vi "set Swept SA - Marker.vi"(6 "On?":bool, 8 "error in (no error)":errorcluster, 9 "trace":i32, 10 "Index":i32, 11 "FSV-40N in":refnum<class "FSV-40N.lvclass">) -> (0 "error out":errorcluster, 3 "FSV-40N out":refnum<class "FSV-40N.lvclass">)   [LabVIEW 2023, in "Spectrum Analyzer.lvlib" / "FSV-40N.lvclass"]
uses:
  FSV-40N.lvclass
  FSV-40N.lvclass/FSV-40N.ctl
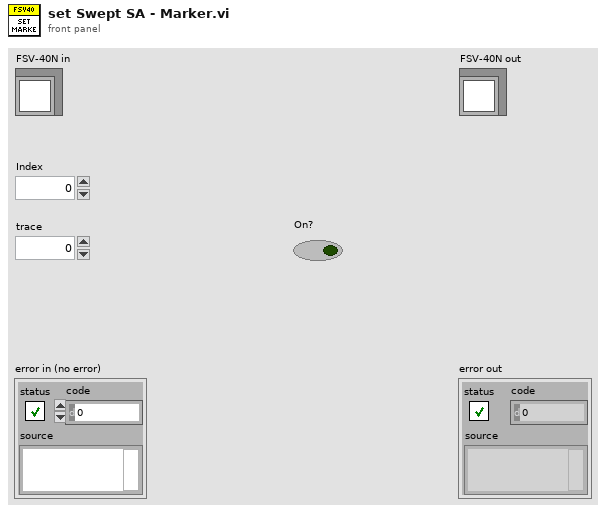
[diagram p1: front panel]
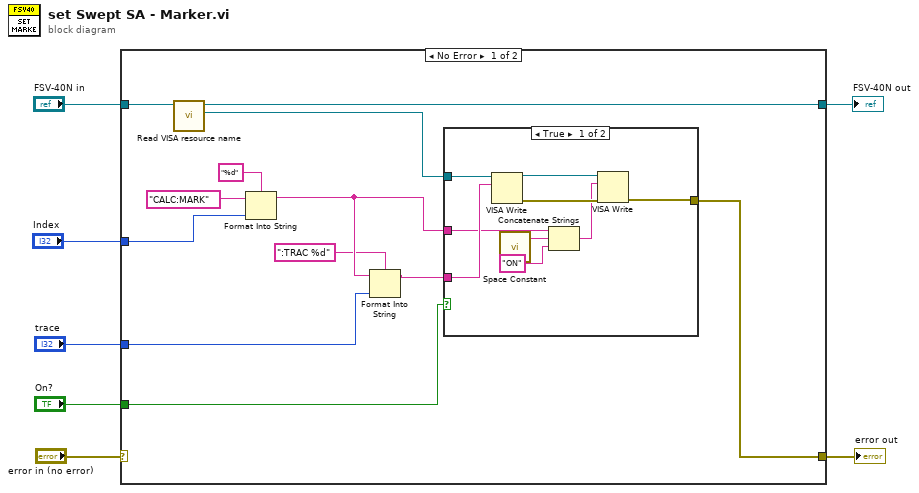
[diagram p0: block diagram]
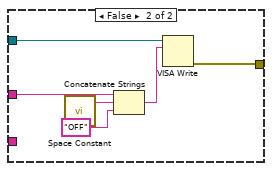
[diagram p2: hidden frame]
diagram:
  n1 = case shown="No Error" "error in (no error)" {
    selector: "error in (no error)" -> [_ w35]
    tunnel: "FSV-40N in" -> [w19 w36]
    tunnel: [w17 w36] -> w5
    tunnel: [w16 w35] -> w4
    tunnel: "Index" -> [w12 _]
    tunnel: "trace" -> [w8 _]
    tunnel: "On?" -> [w15 _]
    frame No Error {
      n2 = call "Read VISA resource name.vi"("FSV-40N in"=w19) -> ("VISA resource name"=w18:refnum<visa-resource-name>, "FSV-40N out"=w17:refnum<class "FSV-40N.lvclass">)  [unwired: 8 in, 1 out]
      n3 = Format Into String(format string="%d", initial string="CALC:MARK" ("string"), w12) -> (resulting string=w11:string)  [unwired: 1 in, 1 out]
      n4 = Format Into String(format string=":TRAC %d" ("string"), initial string=w11, w8) -> (resulting string=w10:string)  [unwired: 1 in, 1 out]
      n5 = case shown="True" w15 {
        tunnel: w18 -> [w28 w34]
        tunnel: [w20 w29] -> w16
        tunnel: w10 -> [w25 _]
        tunnel: w11 -> [w24 w33]
        frame True {
          n6 = VISA Write(VISA resource name=w28, write buffer=w25) -> (VISA resource name out=w27:refnum<visa-resource-name>, error out=w26:errorcluster)  [unwired: 1 in, 1 out]
          n7 = call <vilib>:"Space Constant.vi"() -> ("String"=w23:string)
          n8 = Concatenate Strings(w24, w23, "ON" ("string")) -> (w21:string)
          n9 = VISA Write(VISA resource name=w27, write buffer=w21, error in (no error)=w26) -> (error out=w20:errorcluster)  [unwired: 2 out]
        }
        frame False {
          n10 = call <vilib>:"Space Constant.vi"() -> ("String"=w32:string)
          n11 = Concatenate Strings(w33, w32, "OFF" ("string")) -> (w30:string)
          n12 = VISA Write(VISA resource name=w34, write buffer=w30) -> (error out=w29:errorcluster)  [unwired: 1 in, 2 out]
        }
      }
    }
    frame Error {
    }
  }
  "error out" <- w4
  "FSV-40N out" <- w5
